vi "lvmcp_classname.vi"() -> ()   [LabVIEW 2015]
panel:
  out "error out":errorcluster
  out "class name":string
  in  "reference":refnum<vi>
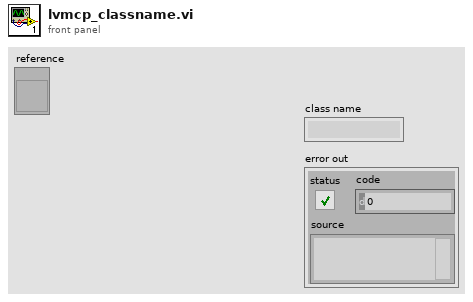
[diagram p1: front panel]
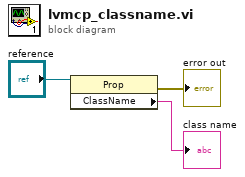
[diagram p0: block diagram]
diagram:
  n1 = property class="Prop"(reference="reference") -> (error out=→"error out":errorcluster, "ClassName"=→"class name":string)  [unwired: 1 in, 1 out]
